vi "Async Action.vi"(8 "error in (no error)":errorcluster, 9 "Message Data":variant, 10 "Message":string, 11 "Application In":refnum<class "Application.lvclass">) -> (0 "error out":errorcluster)   [LabVIEW 2020, in "Application.lvclass"]
doc: "The specific action implemented in the asynchronous action. Multiple different actions may be supported by using the Message and Message Data input to separate them. Any number of actions may run in parallell running the same or different actions. If this method throws an error, the error will be sent to the error handler configured for the process. \nCare needs to be taken so that this action is cancelled if the process is stopped. This may be detected by e.g. observing the Lifecycle: Stopped/Finished broadcast or polling the Get Lifecycle State.vi."
uses:
  Application.lvclass
  Application.lvclass/Application.ctl
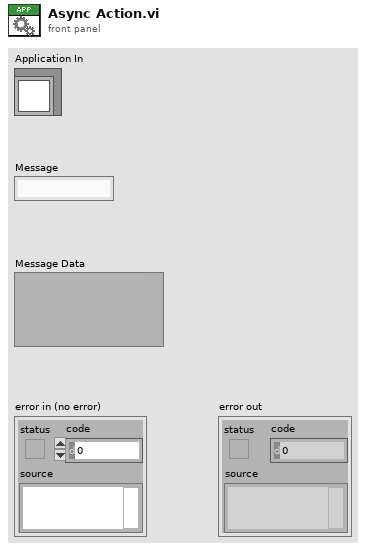
[diagram p1: front panel]
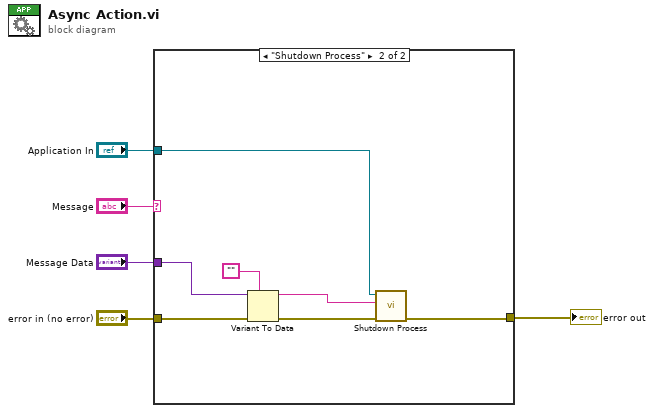
[diagram p0: block diagram]
diagram:
  n1 = case shown="\"Shutdown Process\"" "Message" {
    tunnel: "Application In" -> [_ w9]
    tunnel: "error in (no error)" -> [w6 w13]
    tunnel: [w6 w7] -> w3
    tunnel: "Message Data" -> [_ w12]
    frame Default {
    }
    frame "Shutdown Process" {
      n2 = Variant To Data(error in=w13, type="", Variant=w12) -> (data=w11:string, error out=w8:errorcluster)
      n3 = call "Shutdown Process.vi"("error in (no error)"=w8, "Process Name"=w11, "Application In"=w9) -> ("error out"=w7:errorcluster)  [unwired: 7 in, 1 out]
    }
  }
  "error out" <- w3
